vi "C_Encode_RT.vi"(0 "tx in":u8[](array[numeric]), 1 "brs":bool, 2 "data":u8[](array[numeric]), 5 "id":u32, 7 "ide":bool, 9 "fdf":bool, 11 "error in (no error)":errorcluster) -> (4 "tx out":u8[](array[numeric]), 6 "length":i32, 15 "error out":errorcluster)   [LabVIEW 2021, in "CANsub_C.lvlib"]
doc: "Real-time encode: one CAN or CAN FD frame into a WebSocket frame, written into the caller’s tx buffer (174 bytes, from C_RX_Buffers_Init). No allocation. Send tx bytes 0 … length - 1."
uses:
  CANsub_C.lvlib
  codec_vis/CANsub_Codec.lvlib
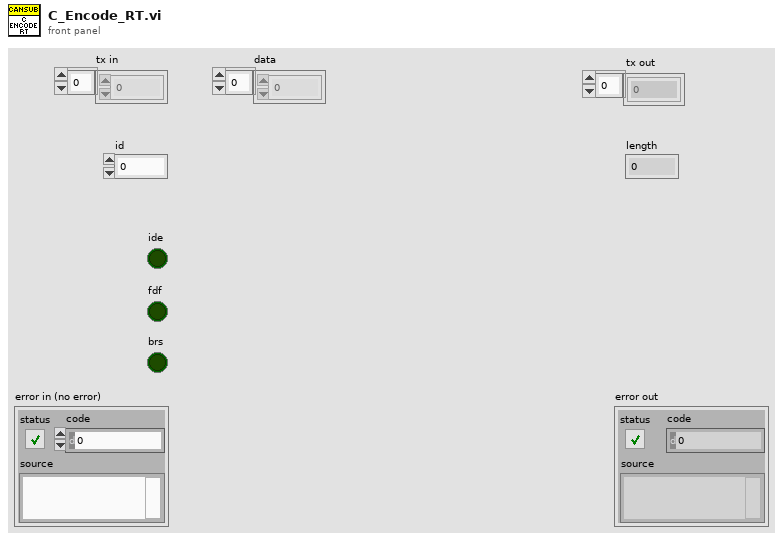
[diagram p1: front panel]
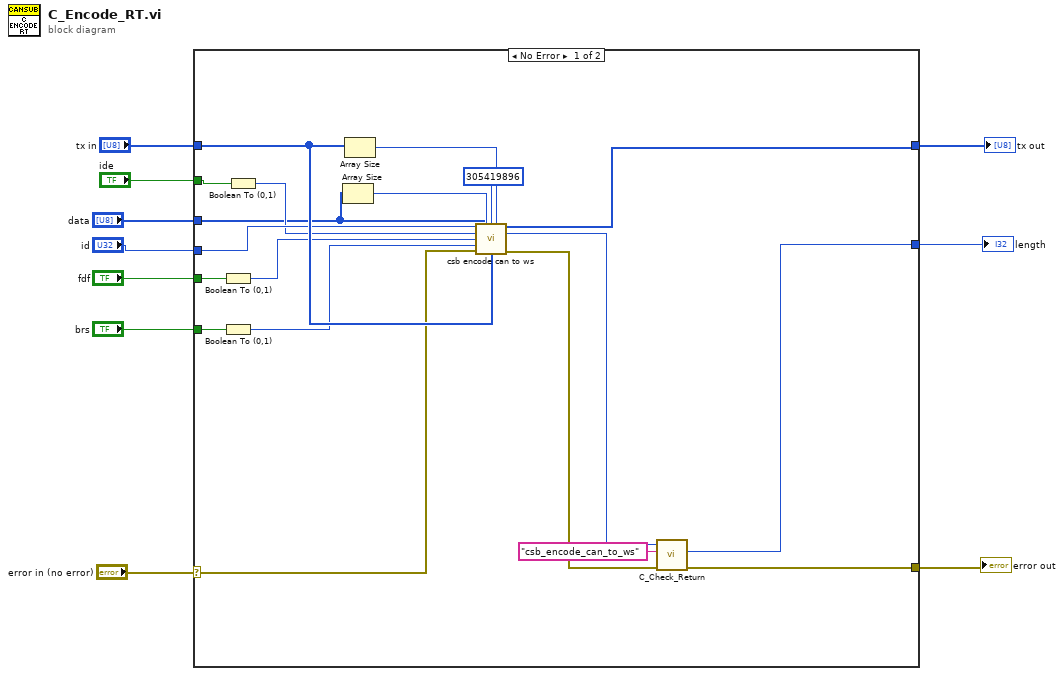
[diagram p0: block diagram]
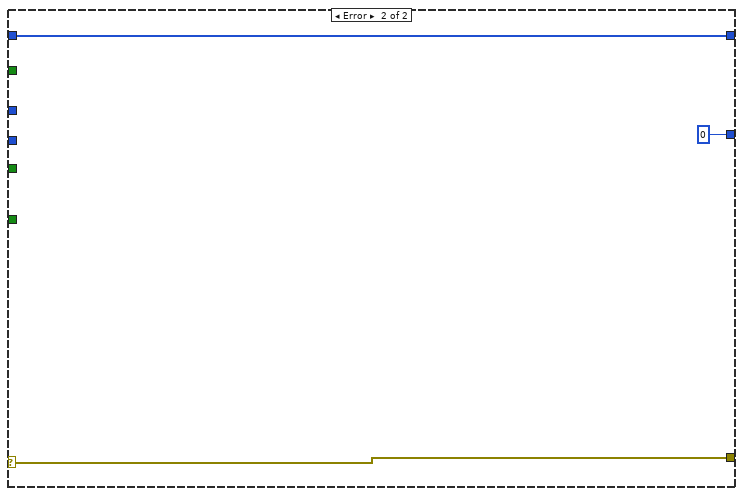
[diagram p2: hidden frame]
diagram:
  n1 = case shown="No Error" "error in (no error)" {
    selector: "error in (no error)" -> [w16 w32]
    tunnel: [w29 w32] -> w9
    tunnel: [w11 w31] -> w8
    tunnel: "tx in" -> [w25 w31]
    tunnel: [w28 0 ("length")] -> w6
    tunnel: "ide" -> [w22 _]
    tunnel: "data" -> [w13 _]
    tunnel: "id" -> [w23 _]
    tunnel: "fdf" -> [w20 _]
    tunnel: "brs" -> [w18 _]
    frame No Error {
      n2 = Boolean To (0,1)(Boolean=w20) -> (0, 1=w19:i16)
      n3 = Boolean To (0,1)(Boolean=w18) -> (0, 1=w17:i16)
      n4 = Boolean To (0,1)(Boolean=w22) -> (0, 1=w21:i16)
      n5 = Array Size(array=w13) -> (size(s)=w14:i32)
      n6 = Array Size(array=w25) -> (size(s)=w24:i32)
      n7 = call "csb encode can to ws.vi"("id"=w23, "data"=w13, "mask"=u32 305419896, "out_cap"=w24, "ide"=w21, "fdf"=w19, "brs"=w17, "error in (no error)"=w16, "len"=w14, "out"=w25) -> ("out out"=w11:u8[], "function return"=w26:i32, "error out"=w15:errorcluster)  [unwired: 3 in]
      n8 = call "C_Check_Return.vi"("error in (no error)"=w15, "function name"="csb_encode_can_to_ws", "function return"=w26) -> ("error out"=w29:errorcluster, "length"=w28:i32)  [unwired: 6 in, 1 out]
    }
    frame Error {
    }
  }
  "tx out" <- w8
  "length" <- w6
  "error out" <- w9
